vi "Initialise Market.vi"() -> (3 "market out":T1)   [LabVIEW 2020, in "Full Featured MCP Server.lvlib"]
doc: "Builds the market state at the start of the server: every stock at its start price, no shares owned, 5000 euros in the wallet. Then simulates 1800 seconds in advance, so the charts and the news list are filled when the first client asks."
uses:
  Full Featured MCP Server.lvlib
  Market State.ctl
  News Item.ctl
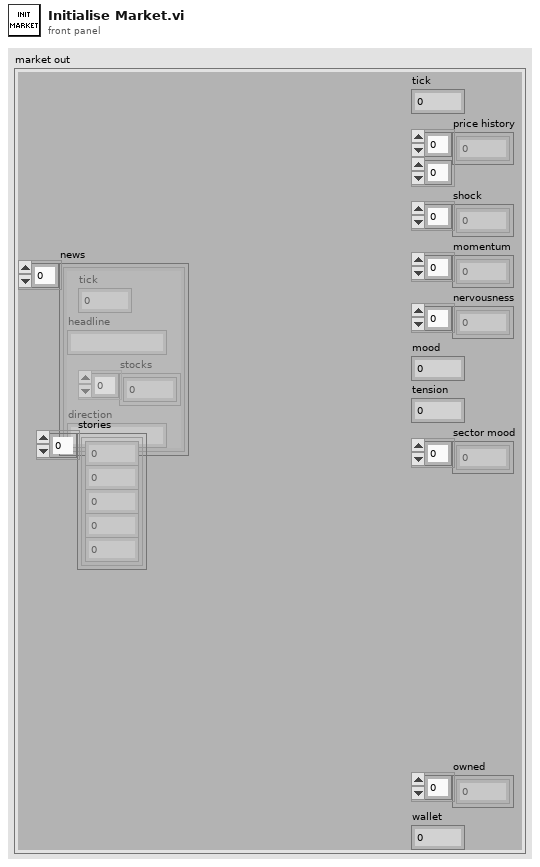
[diagram p1: front panel]
types:
  T1 = typedef "Full Featured MCP Server.lvlib/Market State.ctl" = cluster{"tick":i32, "price history":dbl[][], "shock":dbl[], "momentum":dbl[], "nervousness":dbl[], "mood":dbl, "tension":dbl, "sector mood":dbl[], "news":T2[], "stories":cluster{"arc":i32, "step":i32, "due":i32, "stock":i32, "other":i32}[], "owned":i32[], "wallet":dbl}
  T2 = typedef "Full Featured MCP Server.lvlib/News Item.ctl" = cluster{"tick":i32, "headline":string, "stocks":i32[], "direction":string}
  T3 = cluster{"name":string, "sector":i32, "quality":i32, "start price":dbl, "drift":dbl, "volatility":dbl, "beta":dbl, "jumpiness":dbl, "description":string}[]
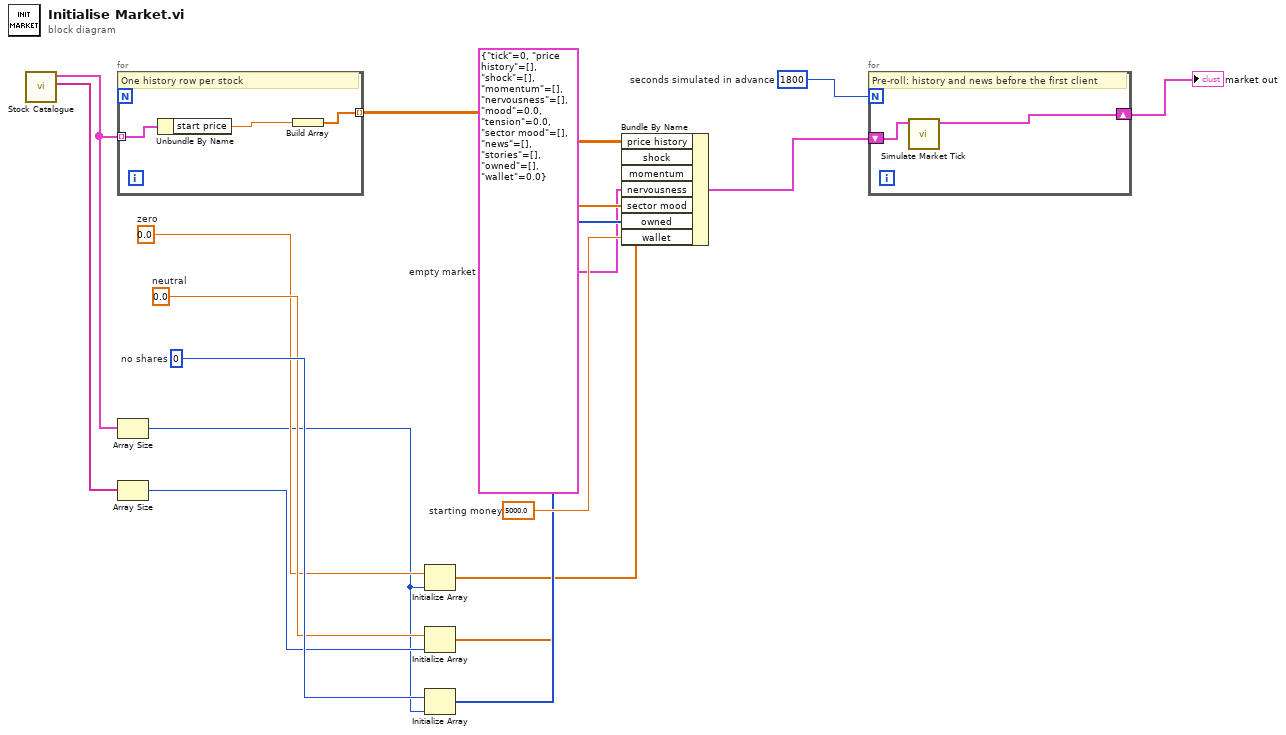
[diagram p0: block diagram]
diagram:
  w15 = 1800  # seconds simulated in advance
  w13 = 5000.0  # starting money
  w11 = 0  # no shares
  w8 = 0.0  # neutral
  w7 = T1 {"tick"=0, "price history"=[], "shock"=[], "momentum"=[], "nervousness"=[], "mood"=0.0, "tension"=0.0, "sector mood"=[], "news"=[], "stories"=[], "owned"=[], "wallet"=0.0}  # empty market
  w5 = 0.0  # zero
  n1 = call "Stock Catalogue.vi"() -> ("sectors"=w2:string[], "stocks"=w1:T3)  [unwired: 10 in]
  n2 = for {
    tunnel: w1 -> [w17] mode=indexing
    tunnel: [w19] -> w3 mode=indexing
    # "One history row per stock"
    n3 = Unbundle By Name(w17) -> ("start price"=w18:dbl)
    n4 = Build Array(w18) -> (w19:dbl[])
  }
  n5 = Array Size(array=w1) -> (size(s)=w4:i32)
  n6 = Array Size(array=w2) -> (size(s)=w9:i32)
  n7 = Initialize Array(w5, w4) -> (w6:dbl[])
  n8 = Initialize Array(w8, w9) -> (w10:dbl[])
  n9 = Initialize Array(w11, w4) -> (w12:i32[])
  n10 = Bundle By Name(cluster=w7, "price history"=w3, "shock"=w6, "momentum"=w6, "nervousness"=w6, "sector mood"=w10, "owned"=w12, "wallet"=w13) -> (w14:T1)
  n11 = for {
    N: w15 -> [_]
    shift-right: [w21] -> w16
    shift-left: w14 -> [w20]
    # "Pre-roll: history and news before the first client"
    n12 = call "Simulate Market Tick.vi"("market"=w20) -> ("market out"=w21:T1)  [unwired: 10 in]
  }
  "market out" <- w16
